vi "Ecrire config LEYBOLD.vi"(2 "error in (no error)":errorcluster caption="entrée d'erreur (pas d'erreur)", 3 "refnum":T1) -> (0 "error out":errorcluster, 1 "refnum out":T1)   [LabVIEW 2022 SP3]
uses:
  <vilib>/Utility/config.llb/Config Data RefNum.ctl
  Variables globales/Variable glob Leybold.vi
  <vilib>/Utility/config.llb/Write Key (String).vi
  <vilib>/Utility/config.llb/Write Key (Boolean).vi
  <vilib>/Utility/config.llb/NI_LVConfig.lvlib
panel:
  out "Noms jauges":string[](array[string])
  out "Ports COM LEYBOLD":refnum<visa-resource-name>[](array[refnum])
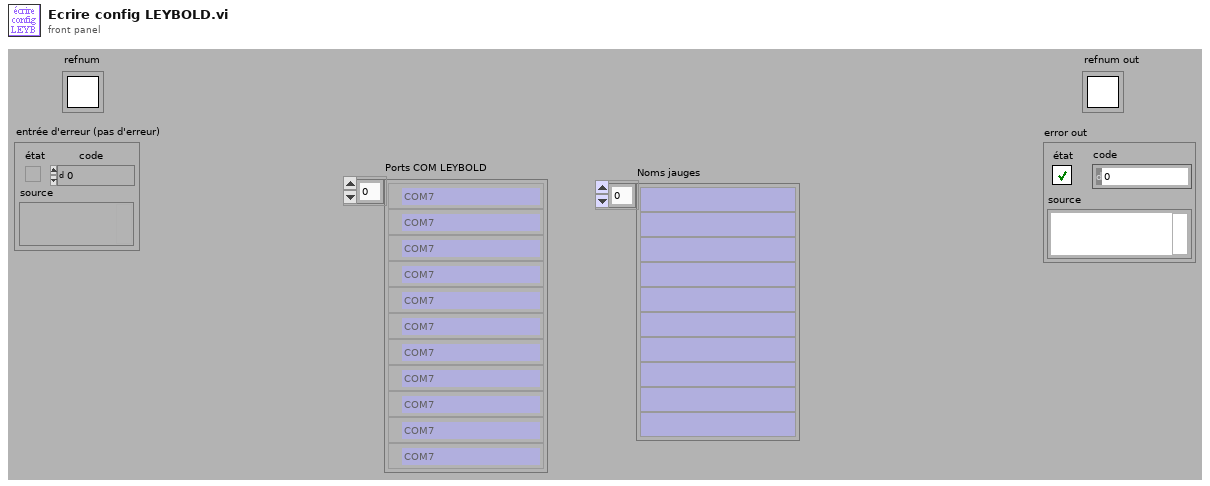
[diagram p1: front panel]
types:
  T1 = typedef "NI_LVConfig.lvlib/Config Data RefNum.ctl" = refnum<k1>
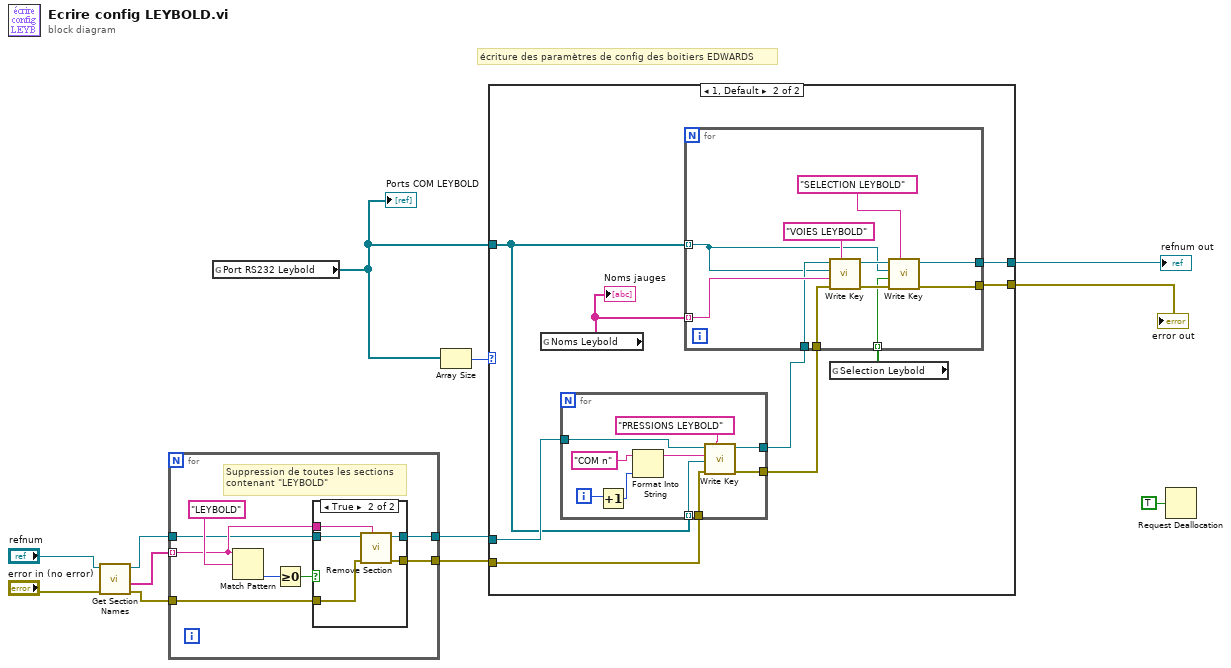
[diagram p0: block diagram]
diagram:
  # "écriture des paramètres de config des boitiers EDWARDS"
  n1 = call <vilib>:"Get Section Names.vi"("error in (no error)"="error in (no error)", "refnum"="refnum") -> ("error out"=w9:errorcluster, "section names"=w7:string[], "refnum out"=w8:T1)  [unwired: 7 in]
  n2 = for {
    tunnel: w7 -> [w17] mode=indexing
    tunnel: w8 -> [w16]
    tunnel: w9 -> [w15]
    tunnel: [w14] -> w4
    tunnel: [w13] -> w3
    # "Suppression de toutes les sections\ncontenant \"LEYBOLD\""
    n3 = Match Pattern(string=w17, regular expression="LEYBOLD" ("expression régulière")) -> (offset past match=w19:i32)  [unwired: 1 in, 3 out]
    n4 = Greater Or Equal To 0?(x=w19) -> (x >= 0?=w18:bool)
    n5 = case shown="True" w18 {
      tunnel: w17 -> [_ w27]
      tunnel: w16 -> [w22 w26]
      tunnel: w15 -> [w21 w25]
      tunnel: [w22 w24] -> w14
      tunnel: [w21 w23] -> w13
      frame False {
      }
      frame True {
        n6 = call <vilib>:"Remove Section.vi"("section"=w27, "error in (no error)"=w25, "refnum"=w26) -> ("error out"=w23:errorcluster, "refnum out"=w24:T1)  [unwired: 6 in, 1 out]
      }
    }
  }
  n7 = global read "Variable glob Leybold.vi" "Port RS232 Leybold"() -> (w2:refnum<visa-resource-name>[])
  "Ports COM LEYBOLD" <- w2
  n8 = Array Size(array=w2) -> (size(s)=w10:i32)
  n9 = case shown="1, Default" w10 {
    tunnel: w3 -> [w28 w38]
    tunnel: w4 -> [w29 w37]
    tunnel: [w29 w34] -> w12
    tunnel: [w28 w33] -> w11
    tunnel: w2 -> [_ w32]
    frame 0 {
    }
    frame 1, Default {
      n10 = global read "Variable glob Leybold.vi" "Noms Leybold"() -> (w31:string[])
      "Noms jauges" <- w31
      n11 = for {
        tunnel: w32 -> [w56] mode=indexing
        tunnel: w37 -> [w54]
        tunnel: w38 -> [w53]
        tunnel: [w52] -> w35
        tunnel: [w51] -> w36
        i -> [w59]
        n12 = Increment(x=w59) -> (x+1=w58:i32)
        n13 = Format Into String(initial string="COM n", w58) -> (resulting string=w57:string)  [unwired: 2 in, 1 out]
        n14 = call-poly <vilib>:"Write Key.vi"("section"="PRESSIONS LEYBOLD", "error in (no error)"=w53, "value"=w56, "key"=w57, "refnum"=w54) -> ("error out"=w51:errorcluster, "refnum out"=w52:T1)  [unwired: 4 in, 1 out]
      }
      n15 = global read "Variable glob Leybold.vi" "Selection Leybold"() -> (w30:bool[])
      n16 = for {
        tunnel: w31 -> [w49] mode=indexing
        tunnel: w35 -> [w48]
        tunnel: w36 -> [w47]
        tunnel: [w46] -> w33
        tunnel: [w45] -> w34
        tunnel: w32 -> [w40] mode=indexing
        tunnel: w30 -> [w39] mode=indexing
        n17 = call-poly <vilib>:"Write Key.vi"("section"="VOIES LEYBOLD", "error in (no error)"=w47, "value"=w49, "key"=w40, "refnum"=w48) -> ("error out"=w42:errorcluster, "refnum out"=w43:T1)  [unwired: 4 in, 1 out]
        n18 = call-poly <vilib>:"Write Key.vi"("section"="SELECTION LEYBOLD", "error in (no error)"=w42, "value"=w39, "key"=w40, "refnum"=w43) -> ("error out"=w46:errorcluster, "refnum out"=w45:T1)  [unwired: 4 in, 1 out]
      }
    }
  }
  "refnum out" <- w12
  "error out" <- w11
  n19 = Request Deallocation(TRUE ("flag")) -> ()
